vi "Mark Harmonic.vi"(8 "error in (no error)":errorcluster caption="에러 입력(에러 없음)", 10 "Fundamental Freq":dbl, 11 "Instrument Manager 입력":refnum<class "Instrument Manager.lvclass">) -> (0 "error out":errorcluster caption="에러 출력", 1 "Frequency":dbl[](array[numeric]), 2 "Amplitude":dbl[](array[numeric]), 3 "Instrument Manager 출력":refnum<class "Instrument Manager.lvclass">)   [LabVIEW 2023, in "Instrument Manager.lvclass"]
uses:
  Instrument Manager.lvclass
  Instrument Manager.lvclass/Instrument Manager.ctl
panel:
  out "배열 2":i32[](array[numeric])
  out "배열":cluster{"Start":dbl, "End":dbl}[](array[cluster])
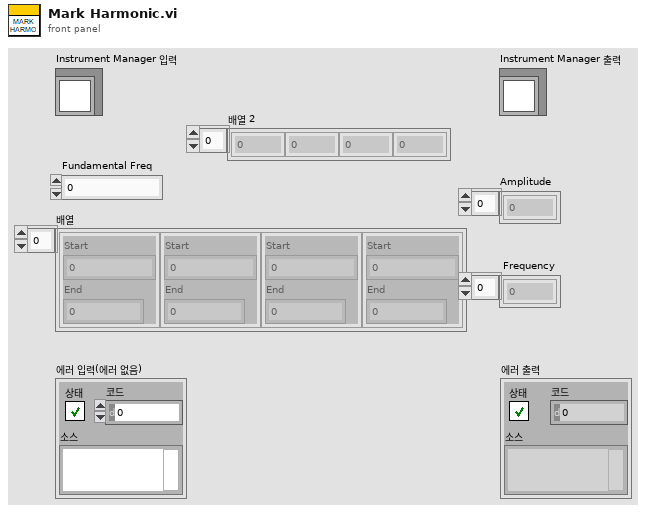
[diagram p1: front panel]
types:
  T1 = typedef "Spectrum Analyzer.lvlib/TYPE Trace Value Array.ctl" = cluster{"Frequency":dbl[], "Amplitude":dbl[]}
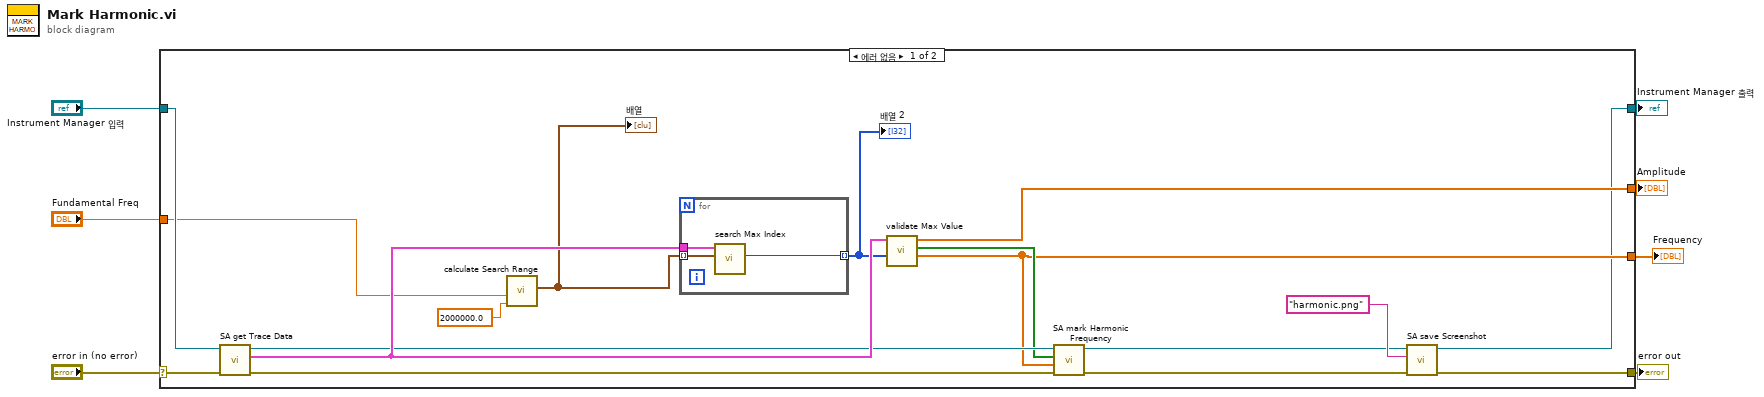
[diagram p0: block diagram]
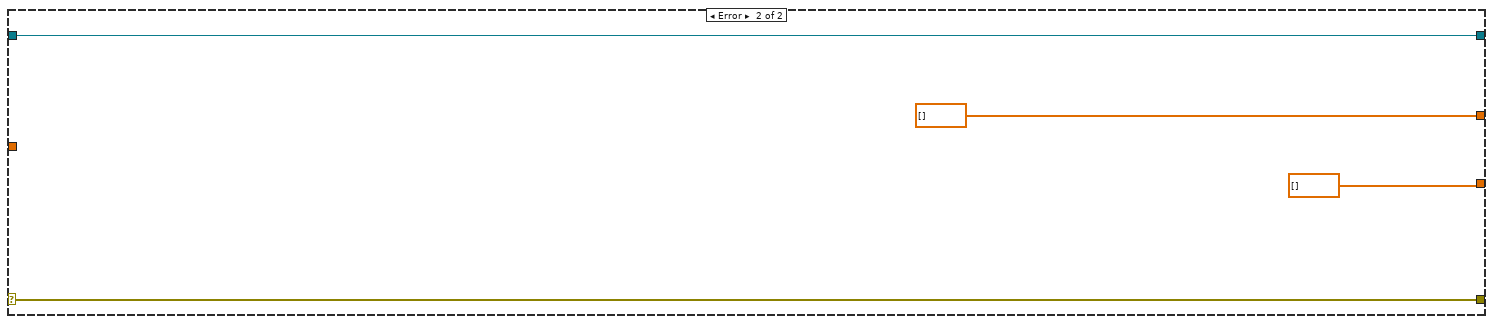
[diagram p2: hidden frame]
diagram:
  n1 = case shown="에러 없음" "error in (no error)" {
    selector: "error in (no error)" -> [w24 w31]
    tunnel: [w10 w31] -> w6
    tunnel: [w8 w30] -> w4
    tunnel: "Instrument Manager 입력" -> [w23 w30]
    tunnel: [w19 dbl[] [] ("Amplitude")] -> w3
    tunnel: "Fundamental Freq" -> [w16 _]
    tunnel: [w13 dbl[] [] ("Frequency")] -> w1
    frame No Error {
      n2 = call "SA get Trace Data.vi"("error in (no error)"=w24, "Instrument Manager 입력"=w23) -> ("error out"=w21:errorcluster, "Trace Values"=w22:T1, "Instrument Manager 출력"=w20:refnum<class "Instrument Manager.lvclass">)  [unwired: 7 in]
      n3 = call "calculate Search Range.vi"("Search Width"=2000000.0, "Fundametal Freq"=w16) -> ("배열"=w15:cluster{"Start":dbl, "End":dbl}[])  [unwired: 9 in]
      "배열" <- w15
      n4 = for {
        tunnel: w15 -> [w27] mode=indexing
        tunnel: w22 -> [w25]
        tunnel: [w26] -> w14 mode=indexing
        n5 = call "search Max Index.vi"("Trace Values"=w25, "Search Range"=w27) -> ("Index"=w26:i32)  [unwired: 8 in]
      }
      "배열 2" <- w14
      n6 = call "validate Max Value.vi"("Max Index"=w14, "Trace Values"=w22) -> ("Frequency"=w13:dbl[], "isExceed?"=w18:bool[], "Amplitude"=w19:dbl[])  [unwired: 7 in]
      n7 = call "SA mark Harmonic Frequency.vi"("error in (no error)"=w21, "Frequency"=w13, "isExceed?"=w18, "Instrument Manager 입력"=w20) -> ("error out"=w11:errorcluster, "Instrument Manager 출력"=w9:refnum<class "Instrument Manager.lvclass">)  [unwired: 6 in]
      n8 = call "SA save Screenshot.vi"("error in (no error)"=w11, "File Name"="harmonic.png", "Instrument Manager 입력"=w9) -> ("error out"=w10:errorcluster, "Instrument Manager 출력"=w8:refnum<class "Instrument Manager.lvclass">)  [unwired: 7 in]
    }
    frame Error {
    }
  }
  "error out" <- w6
  "Instrument Manager 출력" <- w4
  "Amplitude" <- w3
  "Frequency" <- w1
